vi "Copy-Paste.vi"(5 "Copy All (T - Yes)":bool, 7 "Copy/Paste (False, Copy)":bool, 8 "error in (no error)":errorcluster, 11 "Diagram In":refnum<vi>) -> (0 "error out":errorcluster, 3 "Diagram Out":refnum<vi>)   [LabVIEW 2012, in "Scripting Tools.lvlib"]
uses:
  Scripting Tools.lvlib
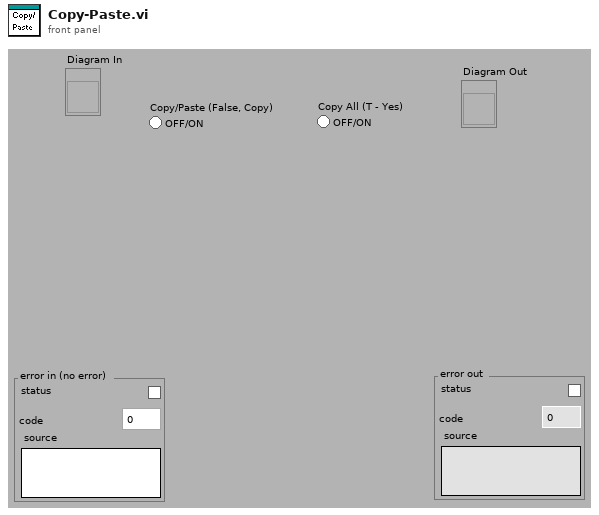
[diagram p1: front panel]
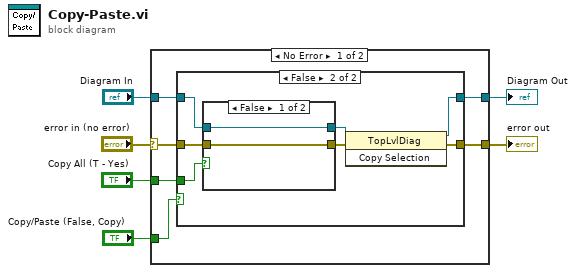
[diagram p0: block diagram]
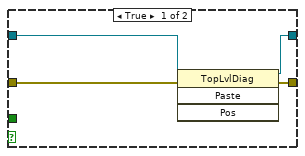
[diagram p2: hidden frame]
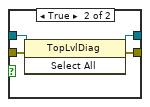
[diagram p3: hidden frame]
diagram:
  n1 = case shown="No Error" "error in (no error)" {
    selector: "error in (no error)" -> [w9 w30]
    tunnel: "Diagram In" -> [w10 w31]
    tunnel: [w12 w30] -> w5
    tunnel: [w11 w31] -> w4
    tunnel: "Copy All (T - Yes)" -> [w8 _]
    tunnel: "Copy/Paste (False, Copy)" -> [w7 _]
    frame No Error {
      n2 = case shown="False" w7 {
        tunnel: [w16 w23] -> w12
        tunnel: [w15 w22] -> w11
        tunnel: w10 -> [w14 w21]
        tunnel: w9 -> [w13 w18]
        tunnel: w8 -> [_ w17]
        frame True {
          n3 = invoke class="TopLvlDiag" method="Paste"(reference=w14, error in=w13) -> (reference out=w15:refnum<vi>, error out=w16:errorcluster)  [unwired: 2 in, 2 out]
        }
        frame False {
          n4 = case shown="False" w17 {
            tunnel: w21 -> [w25 w29]
            tunnel: [w25 w27] -> w20
            tunnel: [w24 w26] -> w19
            tunnel: w18 -> [w24 w28]
            frame False {
            }
            frame True {
              n5 = invoke class="TopLvlDiag" method="Select All"(reference=w29, error in=w28) -> (reference out=w27:refnum<vi>, error out=w26:errorcluster)  [unwired: 1 in, 1 out]
            }
          }
          n6 = invoke class="TopLvlDiag" method="Copy Selection"(reference=w20, error in=w19) -> (reference out=w22:refnum<vi>, error out=w23:errorcluster)  [unwired: 1 in, 1 out]
        }
      }
    }
    frame Error {
    }
  }
  "error out" <- w5
  "Diagram Out" <- w4
